vi "Server Send Queue.vi"(11 "创建?":bool) -> (0 "error out":errorcluster caption="错误输出", 3 "上传队列":refnum<queue>)   [LabVIEW 2020, in "TCP Communication.lvlib"]
uses:
  TCP Communication.lvlib
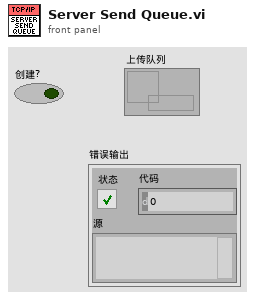
[diagram p1: front panel]
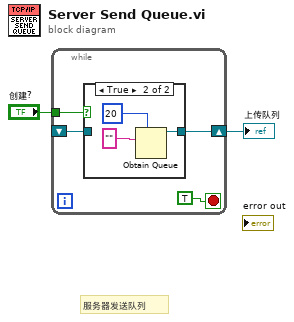
[diagram p0: block diagram]
diagram:
  # "服务器发送队列"
  n1 = while {
    shift-right: [w6] -> w2
    shift-left: _ -> [w3]
    tunnel: "创建?" -> [w4]
    stop <- TRUE stop-if-true
    n2 = case shown="True" w4 {
      tunnel: [w7 w9] -> w6
      tunnel: w3 -> [w7 _]
      frame False {
      }
      frame True {
        n3 = Obtain Queue(max queue size (-1, unlimited)=20 ("队列最大值（-1，无限）"), element data type="") -> (queue out=w9:refnum<queue>)  [unwired: 3 in, 2 out]
      }
    }
  }
  "上传队列" <- w2
